vi "Own20261012_PublicGetObjectPosition.vi"() -> ()   [LabVIEW 2024]
uses:
  <vilib>/Utility/miscctls.llb/LVPositionTypeDef.ctl
panel:
  out "error out":errorcluster caption="错误输出"
  out "position":T1 caption="位置"
  in  "object_id":u32
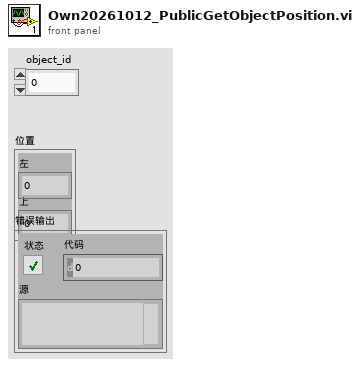
[diagram p1: front panel]
types:
  T1 = typedef "LVPositionTypeDef.ctl" = cluster{"Left":i32, "Top":i32}
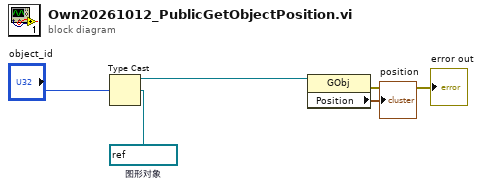
[diagram p0: block diagram]
diagram:
  w4 = refnum<vi> refnum  # 图形对象
  n1 = Type Cast ("强制类型转换")(type=w4, x="object_id") -> (*(type *) &x=w3:refnum<vi>)
  n2 = property on="属性节点" class="GObj"(reference=w3) -> (error out=→"error out":errorcluster, "Position"=→"position":T1)  [unwired: 1 in, 1 out]
